vi "[ex ce] Eval X-Y(t).vi"() -> ()   [LabVIEW 2021]
doc: "CE-Math example.\n\n::: CalcExpress Toolkit :::\nCopyright (c) 2000-2026 Konstantin Shifershteyn. All rights reserved."
uses:
  ce exmpl - 1D difference info.ctl
  <vilib>/gmath/NI_Gmath.lvlib
panel:
  out "Y max difference":T1={"index"=-1, "absolute difference"=0.0, "relative difference, %"=0.0} {"relative difference, %" format="%#.6g"; "absolute difference" format="%#.6g"}
  out "X max difference":T1={"index"=-1, "absolute difference"=0.0, "relative difference, %"=0.0} {"relative difference, %" format="%#.6g"; "absolute difference" format="%#.6g"}
  in  "formulas info":T2={"formula 1"="t * sin(a*t)", "formula 2"="b * sqrt(t) * cos(a*t)", "variable"="t"}
  in  "end":dbl=10.0 format="%.2f"
  in  "start":dbl format="%.2f"
  out "speed ratio":dbl format="%.3f"
  out "GM ticks":u32 caption="ms"
  out "CE ticks":u32 caption="ms"
  out "CE Graph":cluster{"X(t)":dbl[], "Y(t)":dbl[]}(graph) caption="CalcExpress"
  in  "# points":u32=1000
  in  "parameters":cluster{"name":string, "value":dbl}[](array[cluster])=[{"name"="a", "value"=3.0}, {"name"="b", "value"=6.0}] {"value" format="%.2f"}
  out "GM Graph":cluster{"X(t)":dbl[], "Y(t)":dbl[]}(graph) caption="G Math"
  # "NOTE    CalcExpress uses (^) operator to perform bitwise-XOR operation but\nnot exponentiation operation. You have to use double-asterisk (**) operator\nto compute an exponent in a CalcExpress expression. For sample, x**y ."
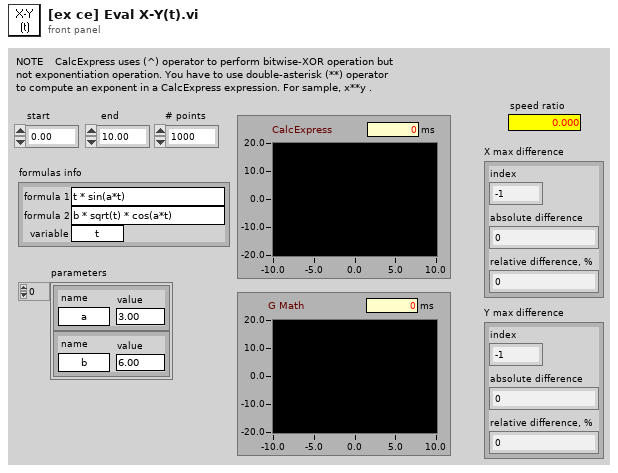
[diagram p1: front panel]
types:
  T1 = typedef "ce exmpl - 1D difference info.ctl" = cluster{"index":i32, "absolute difference":dbl, "relative difference, %":dbl}
  T2 = cluster{"formula 1":string, "formula 2":string, "variable":string}
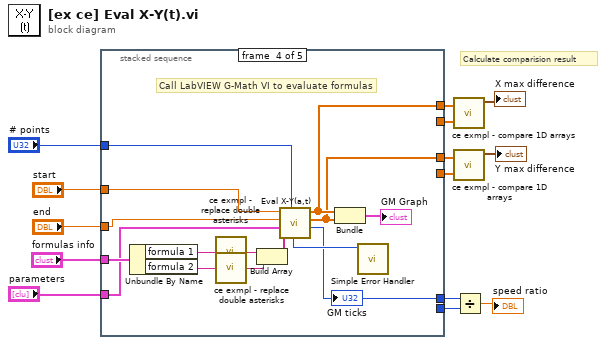
[diagram p0: block diagram]
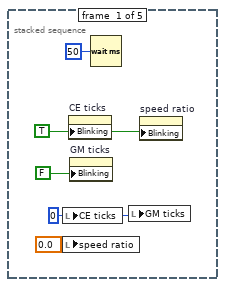
[diagram p2: hidden frame]
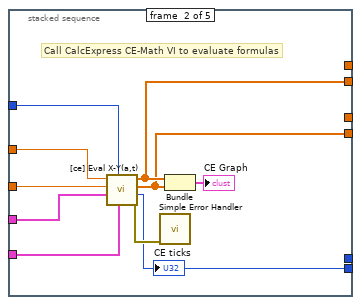
[diagram p3: hidden frame]
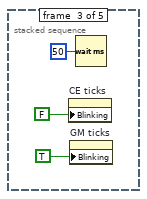
[diagram p4: hidden frame]
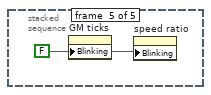
[diagram p5: hidden frame]
diagram:
  # "Calculate comparision result"
  n1 = stacked-sequence {
    tunnel: "start" -> [_ w27 _ w41 _]
    tunnel: "end" -> [_ w26 _ w42 _]
    tunnel: "formulas info" -> [_ w25 _ w45 _]
    tunnel: "parameters" -> [_ w24 _ w44 _]
    tunnel: "# points" -> [_ w23 _ w46 _]
    tunnel: [_ w28 _ _ _] -> w12
    tunnel: [_ _ _ w43 _] -> w10
    tunnel: [_ _ _ w38 _] -> w6
    tunnel: [_ w21 _ _ _] -> w5
    tunnel: [_ w20 _ _ _] -> w4
    tunnel: [_ _ _ w37 _] -> w3
    frame #0 {
      w16 = u32 0 ("CE ticks")
      w18 = TRUE ("Write Attribute")
      n2 = local write "CE ticks"(w16) -> ()
      n3 = local write "speed ratio"(0.0 ("speed ratio")) -> ()
      n4 = property on="CE ticks" class="DigNum (strict)"("Blinking"=w18) -> ()  [unwired: 2 in, 2 out]
      n5 = property on="GM ticks" class="DigNum (strict)"("Blinking"=FALSE ("Write Attribute")) -> ()  [unwired: 2 in, 2 out]
      n6 = Wait (ms)(milliseconds to wait=u32 50) -> ()  [unwired: 1 out]
      n7 = local write "GM ticks"(w16) -> ()
      n8 = property on="speed ratio" class="DigNum (strict)"("Blinking"=w18) -> ()  [unwired: 2 in, 2 out]
    }
    frame #1 {
      # "Call CalcExpress CE-Math VI to evaluate formulas"
      n9 = call "[ce] Eval X-Y(a,t).vi"("parameters"=w24, "# points"=w23, "formulas info"=w25, "end"=w26, "start"=w27) -> ("error out"=w29:errorcluster, "ticks"=w28:u32, "Y"=w20:dbl[], "X"=w21:dbl[])  [unwired: 3 in]
      "CE ticks" <- w28
      n10 = call <vilib>:"Simple Error Handler.vi"("error in (no error)"=w29) -> ()  [unwired: 4 in, 5 out]
      n11 = Bundle("X"=w21, "Y"=w20) -> (→"CE Graph":cluster{"X":dbl[], "Y":dbl[]})  [unwired: 1 in]
    }
    frame #2 {
      n12 = property on="CE ticks" class="DigNum (strict)"("Blinking"=FALSE ("Write Attribute")) -> ()  [unwired: 2 in, 2 out]
      n13 = property on="GM ticks" class="DigNum (strict)"("Blinking"=TRUE ("Write Attribute")) -> ()  [unwired: 2 in, 2 out]
      n14 = Wait (ms)(milliseconds to wait=u32 50) -> ()  [unwired: 1 out]
    }
    frame #3 {
      # "Call LabVIEW G-Math VI to evaluate formulas"
      n15 = Unbundle By Name(w45) -> ("formula 1"=w36:string, "formula 2"=w35:string)
      n16 = call "ce exmpl - replace double asterisks .vi"("formula in"=w36) -> ("formula out"=w34:string)  [unwired: 4 in]
      n17 = call "ce exmpl - replace double asterisks .vi"("formula in"=w35) -> ("formula out"=w33:string)  [unwired: 4 in]
      n18 = Build Array(w34, w33) -> (w40:string[])
      n19 = call <vilib>:"Eval X-Y(a,t).vi"("number of points"=w46, "Formulas"=w40, "Parameters"=w44, "end"=w42, "start"=w41) -> ("error"=w47:i32, "ticks"=w43:u32, "Y"=w37:dbl[], "X"=w38:dbl[])
      "GM ticks" <- w43
      n20 = Bundle("X"=w38, "Y"=w37) -> (→"GM Graph":cluster{"X":dbl[], "Y":dbl[]})  [unwired: 1 in]
      n21 = call <vilib>:"Simple Error Handler.vi"("error code (no error:0)"=w47) -> ()  [unwired: 4 in, 5 out]
    }
    frame #4 {
      w48 = FALSE ("Write Attribute")
      n22 = property on="GM ticks" class="DigNum (strict)"("Blinking"=w48) -> ()  [unwired: 2 in, 2 out]
      n23 = property on="speed ratio" class="DigNum (strict)"("Blinking"=w48) -> ()  [unwired: 2 in, 2 out]
    }
  }
  n24 = call "ce exmpl - compare 1D arrays.vi"("checking array B"=w5, "standard array A"=w6) -> ("max absolute difference"=→"X max difference":T1)  [unwired: 1 in, 3 out]
  n25 = call "ce exmpl - compare 1D arrays.vi"("checking array B"=w4, "standard array A"=w3) -> ("max absolute difference"=→"Y max difference":T1)  [unwired: 1 in, 3 out]
  n26 = Divide(x=w10, y=w12) -> (x/y=→"speed ratio":dbl)
